vi "Initialize Stores.vi"(8 "error in":errorcluster, 11 "Data Folder":path) -> (0 "error out":errorcluster, 2 "Entry Running?":bool, 3 "Running Entry":T1, 4 "Time Entry Store out":refnum<class "Time Entry Store.lvclass">, 5 "Project Store out":refnum<class "Project Store.lvclass">)   [LabVIEW 2026]
doc: "Opens the application's storage at startup. An empty Data Folder (or Not a Path) means %LOCALAPPDATA%\\LVTimeTracker, the folder the INI classes have always used; the folder is created when it does not exist. Version-1 data in it is migrated first (Migrate v1 Data.vi backs it up and does nothing when the folder is already schema version 2). Then a Project Store-INI and a Time Entry Store-INI are created and initialized on the folder, the projects and tasks are read, and the running entry is looked up.\n\nInputs: Data Folder; error in.\nOutputs: Running Entry (the running time entry, a default row with an empty ID when nothing is running); Entry Running?; Project Store out (a Project Store-INI, already read); Time Entry Store out (a Time Entry Store-INI); error out.\n\nGenerated by: Claude"
uses:
  Storage/Rows/Time Entry.ctl
  Storage/Project Store/Project Store.lvclass
  Storage/Time Entry Store/Time Entry Store.lvclass
  Storage/Project Store-INI/Project Store-INI.lvclass
  Storage/Time Entry Store-INI/Time Entry Store-INI.lvclass
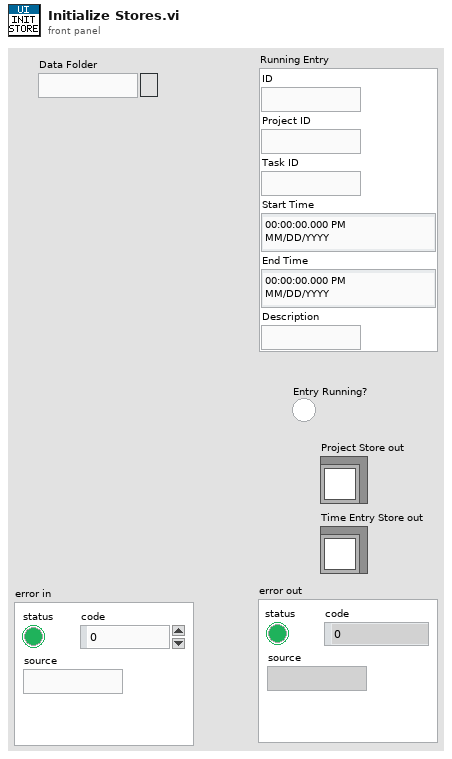
[diagram p1: front panel]
types:
  T1 = typedef "Time Entry.ctl" = cluster{"ID":string, "Project ID":string, "Task ID":string, "Start Time":timestamp, "End Time":timestamp, "Description":string}
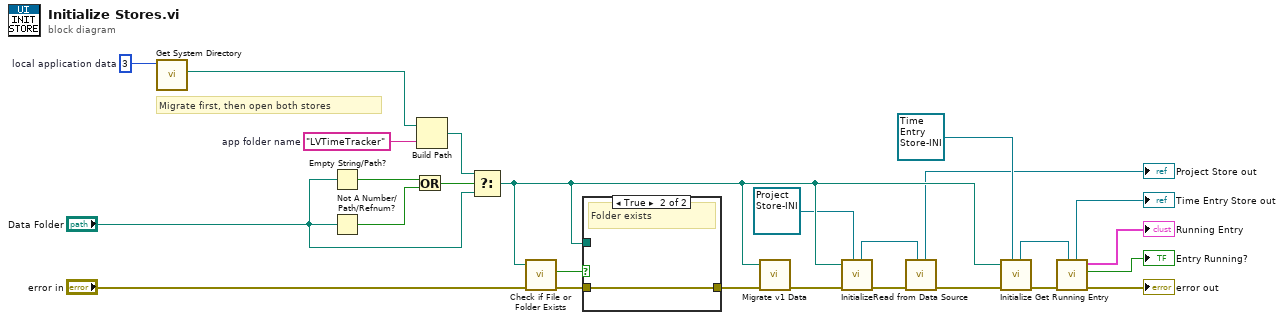
[diagram p0: block diagram]
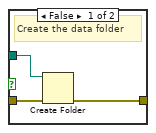
[diagram p2: hidden frame]
diagram:
  w9 = "LVTimeTracker"  # app folder name
  w8 = 3  # local application data
  # "Migrate first, then open both stores"
  n1 = call <vilib>:"Get System Directory.vi"("system directory type"=w8) -> ("system directory"=w15:path)  [unwired: 10 in]
  n2 = Empty String/Path?(string/path="Data Folder") -> (empty?=w12:bool)
  n3 = Not A Number/Path/Refnum?(number/path/refnum="Data Folder") -> (NaN/Path/Refnum?=w13:bool)
  n4 = Or(x=w12, y=w13) -> (x .or. y?=w14:bool)
  n5 = Build Path(base path=w15, name or relative path=w9) -> (appended path=w16:path)
  n6 = Select(t=w16, s=w14, f="Data Folder") -> (s? t:f=w17:path)
  n7 = call <vilib>:"Check if File or Folder Exists.vi"("error in (no error)"="error in", "path"=w17) -> ("error out"=w19:errorcluster, "file or folder exists?"=w18:bool)  [unwired: 7 in, 1 out]
  n8 = case shown="True" w18 {
    tunnel: w17 -> [w27 _]
    tunnel: w19 -> [w28 w30]
    tunnel: [w29 w30] -> w20
    frame False {
      # "Create the data folder"
      n9 = Create Folder(path (use dialog)=w27, error in=w28) -> (error out=w29:errorcluster)  [unwired: 1 in, 2 out]
    }
    frame True {
      # "Folder exists"
    }
  }
  n10 = call "Migrate v1 Data.vi"("error in (no error)"=w20, "Data Folder"=w17) -> ("error out"=w21:errorcluster)  [unwired: 8 in, 1 out]
  n11 = call-dynamic "Initialize.vi"("Project Store in"=refnum<class "Project Store-INI.lvclass"> refnum ("Project Store-INI"), "error in (no error)"=w21, "Data Folder"=w17) -> ("error out"=w23:errorcluster, "Project Store out"=w22:refnum<class "Project Store-INI.lvclass">)  [unwired: 7 in]
  n12 = call-dynamic "Read from Data Source.vi"("Project Store in"=w22, "error in (no error)"=w23) -> ("error out"=w24:errorcluster, "Project Store out"=→"Project Store out":refnum<class "Project Store-INI.lvclass">)  [unwired: 8 in]
  n13 = call-dynamic "Initialize.vi"("Time Entry Store in"=refnum<class "Time Entry Store-INI.lvclass"> refnum ("Time Entry Store-INI"), "error in (no error)"=w24, "Data Folder"=w17) -> ("error out"=w26:errorcluster, "Time Entry Store out"=w25:refnum<class "Time Entry Store-INI.lvclass">)  [unwired: 7 in]
  n14 = call-dynamic "Get Running Entry.vi"("Time Entry Store in"=w25, "error in (no error)"=w26) -> ("error out"=→"error out":errorcluster, "found?"=→"Entry Running?":bool, "Time Entry"=→"Running Entry":T1, "Time Entry Store out"=→"Time Entry Store out":refnum<class "Time Entry Store-INI.lvclass">)  [unwired: 6 in]
